vi "RemoteVI Encode Popups.vi"(0 "popups":T1(array[cluster]), 5 "origin x":i32, 7 "origin y":i32) -> (4 "overlay popups":cluster{"x":i16, "y":i16, "png":string}[](array[cluster]))   [LabVIEW 2020, in "RemoteVI.lvlib"]
doc: "Captures each popup window (RemoteVI Capture Window.vi - PrintWindow, so hidden, covered or off-screen popups are captured too), PNG-encodes it (RemoteVI Encode Rect PNG.vi) and places it at its window position minus origin, bottom-most first (popups is ordered top-most first, so it is walked from the end). A popup whose capture or encoding failed is left out. The result is the input of RemoteVI Overlay Encode.vi (docs\\protocol.md section 3.2)."
uses:
  RemoteVI.lvlib
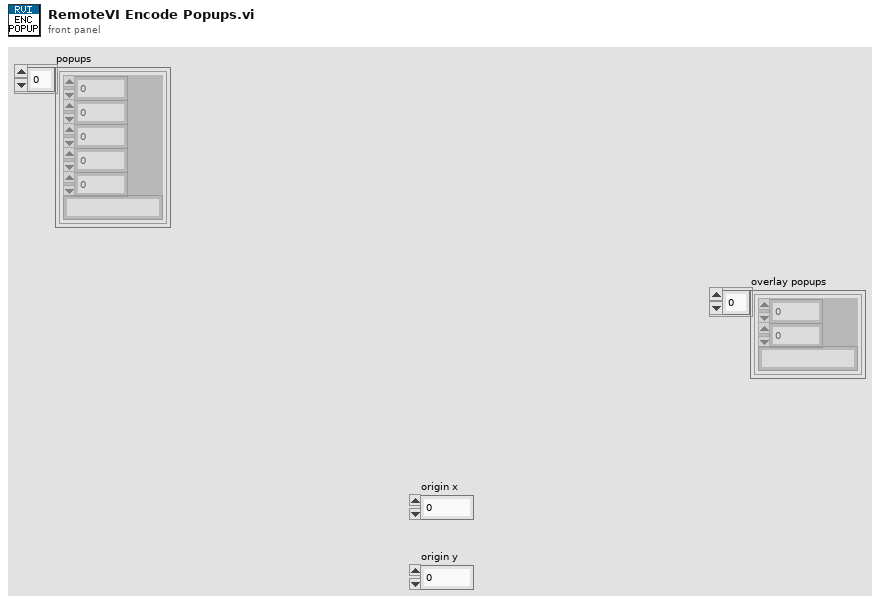
[diagram p1: front panel]
types:
  T1 = cluster{"hwnd":u64, "x":i32, "y":i32, "w":i32, "h":i32, "class":string}[]
  T2 = cluster{"hwnd":u64, "x":i32, "y":i32, "w":i32, "h":i32, "class":string}
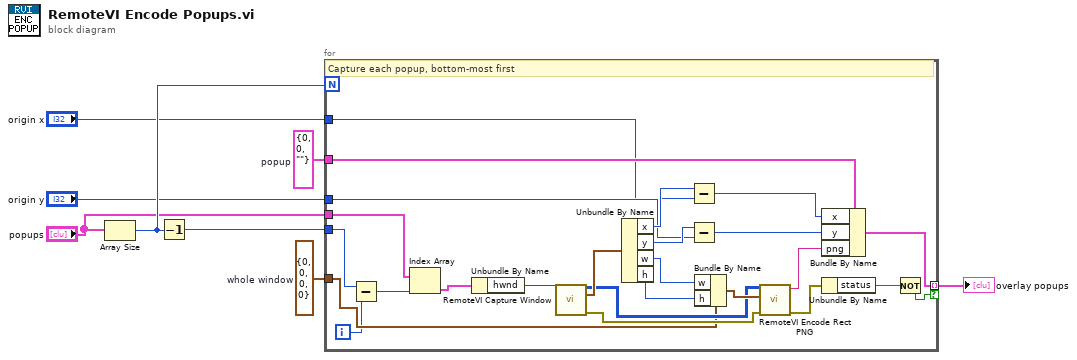
[diagram p0: block diagram]
diagram:
  w7 = cluster{"x":i16, "y":i16, "png":string} {"x"=0, "y"=0, "png"=""}  # popup
  w6 = cluster{"x":i32, "y":i32, "w":i32, "h":i32} {"x"=0, "y"=0, "w"=0, "h"=0}  # whole window
  n1 = Array Size(array="popups") -> (size(s)=w4:i32)
  n2 = Decrement(x=w4) -> (x-1=w5:i32)
  n3 = for {
    N: w4 -> [_]
    tunnel: "popups" -> [w10]
    tunnel: "origin x" -> [w12]
    tunnel: "origin y" -> [w13]
    tunnel: w6 -> [w14]
    tunnel: w7 -> [w15]
    tunnel: w5 -> [w11]
    tunnel: [w31] -> w8 mode=indexing if=w33
    i -> [w9]
    # "Capture each popup, bottom-most first"
    n4 = Subtract(x=w11, y=w9) -> (x-y=w16:i32)
    n5 = Index Array(array=w10, index=w16) -> (element=w17:T2)
    n6 = Unbundle By Name(w17) -> ("hwnd"=w18:u64)
    n7 = call "RemoteVI Capture Window.vi"("hwnd"=w18) -> ("pixmap"=w19:u32[][], "rect"=w20:cluster{"x":i32, "y":i32, "w":i32, "h":i32}, "error out"=w21:errorcluster)  [unwired: 12 in]
    n8 = Unbundle By Name(w20) -> ("x"=w22:i32, "y"=w23:i32, "w"=w24:i32, "h"=w25:i32)
    n9 = Subtract(x=w22, y=w12) -> (x-y=w29:i32)
    n10 = Subtract(x=w23, y=w13) -> (x-y=w30:i32)
    n11 = Bundle By Name(cluster=w14, "w"=w24, "h"=w25) -> (w26:cluster{"x":i32, "y":i32, "w":i32, "h":i32})
    n12 = call "RemoteVI Encode Rect PNG.vi"("error in"=w21, "rect"=w26, "pixmap"=w19) -> ("error out"=w28:errorcluster, "png"=w27:string)  [unwired: 7 in]
    n13 = Bundle By Name(cluster=w15, "x"=w29, "y"=w30, "png"=w27) -> (w31:cluster{"x":i16, "y":i16, "png":string})
    n14 = Unbundle By Name(w28) -> ("status"=w32:bool)
    n15 = Not(x=w32) -> (.not. x?=w33:bool)
  }
  "overlay popups" <- w8
